vi "KY DeviceDisplayName.vi"(8 "error in (no error)":errorcluster, 11 "index":u32) -> (0 "error out":errorcluster, 3 "function return":string)   [LabVIEW 2023, in "KYFGLib_lv.lvlib"]
doc: "KYFG_API const char* KYFG_Pid2Name(unsigned int pid);"
uses:
  KYFGLib_lv.lvlib
  KYFGLib.dll
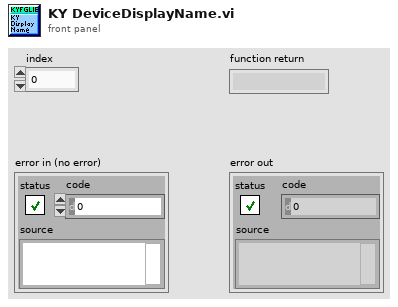
[diagram p1: front panel]
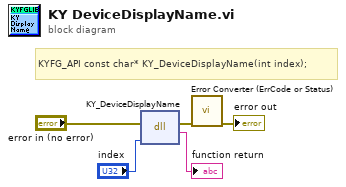
[diagram p0: block diagram]
diagram:
  # "KYFG_API const char* KY_DeviceDisplayName(int index);"
  n1 = dll-call lib="KYFGLib.dll" fn="KY_DeviceDisplayName"(error in="error in (no error)", "index"="index") -> (error out=w3:errorcluster, "return type"=→"function return":string)  [unwired: 3 in, 1 out]
  n2 = call "Error Converter (ErrCode or Status).vi"("error in (no error)"=w3) -> ("error out"=→"error out":errorcluster)  [unwired: 10 in]
